vi "RFH-read_folder-common_format.vi"(7 "File Path":path, 8 "error In":errorcluster) -> (0 "error out":errorcluster, 1 "Data":T1[](array[typedef]), 2 "Names":string[](array[string]))   [LabVIEW 2020, in "RFH-Reflection_File_Handler.lvlib"]
doc: "Reads every common-format file in a folder. Returns the data and the file names without extension."
uses:
  RFH-Reflection_File_Handler.lvlib
  RFH-common_data_format.ctl
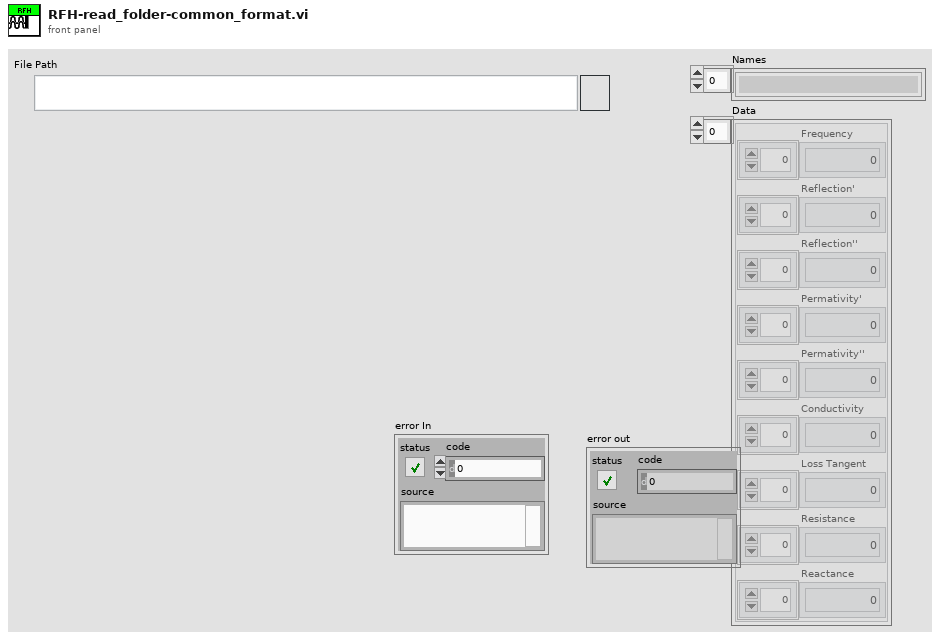
[diagram p1: front panel]
types:
  T1 = typedef "RFH-Reflection_File_Handler.lvlib/RFH-common_data_format.ctl" = cluster{"Frequency":dbl[], "Reflection'":dbl[], "Reflection''":dbl[], "Permativity'":dbl[], "Permativity''":dbl[], "Conductivity":dbl[], "Loss Tangent":dbl[], "Resistance":dbl[], "Reactance":dbl[]}
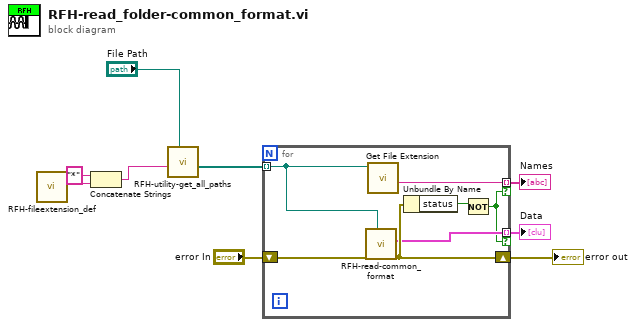
[diagram p0: block diagram]
diagram:
  n1 = call "RFH-fileextension_def.vi"() -> ("File extention"=w4:string)  [unwired: 10 in, 1 out]
  n2 = Concatenate Strings("*" ("string"), w4) -> (w2:string)
  n3 = call "RFH-utility-get_all_paths.vi"("Folder Path"="File Path", "pattern"=w2) -> ("All Files in Dir"=w9:path[])  [unwired: 6 in, 3 out]
  n4 = for {
    tunnel: w9 -> [w15] mode=indexing
    tunnel: [w16] -> w7 mode=indexing if=w10
    shift-right: [w13] -> w5
    shift-left: "error In" -> [w14]
    tunnel: [w11] -> w6 mode=indexing if=w10
    n5 = call "RFH-read-common_format.vi"("file path (dialog if empty)"=w15, "error in"=w14) -> ("error out"=w13:errorcluster, "Common Format"=w11:T1)  [unwired: 8 in]
    n6 = call <vilib>:"Get File Extension.vi"("file"=w15) -> ("filename without extension"=w16:string)  [unwired: 6 in, 4 out]
    n7 = Unbundle By Name(w13) -> ("status"=w12:bool)
    n8 = Not(x=w12) -> (.not. x?=w10:bool)
  }
  "Names" <- w7
  "Data" <- w6
  "error out" <- w5
